vi "Stop server indep.vi"() -> ()   [LabVIEW 2020, in "LabVIEW-Python TCP Lib.lvlib"]
uses:
  LabVIEW-Python TCP Lib.lvlib
panel:
  in  "port":u16=5000
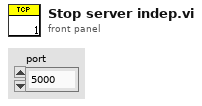
[diagram p1: front panel]
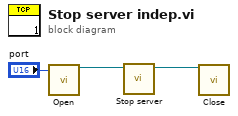
[diagram p0: block diagram]
diagram:
  n1 = call "Open.vi"("port"="port") -> ("connection ID"=w3:refnum<k5>)  [unwired: 9 in, 1 out]
  n2 = call "Stop server.vi"("connection ID"=w3) -> ("connection ID out"=w2:refnum<k5>)  [unwired: 8 in, 2 out]
  n3 = call "Close.vi"("connection ID"=w2) -> ()  [unwired: 9 in, 2 out]
